vi "temperature control.vi"() -> ()   [LabVIEW 2026]
uses:
  <vilib>/Analysis/baseanly.llb/Mean (DBL).vi
  <vilib>/Instr/_visa.llb/VISA Configure Serial Port (Instr).vi
  <vilib>/Analysis/NI_AALBase.lvlib
panel:
  out "Event Log":string
  out "Alarm":bool
  out "Trend":cluster{dbl, "mean":dbl}(graph)
  out "Raw ADC":dbl
  out "Temperature °C":dbl(slide) scale=0.0..100.0
  in  "stop":bool
  in  "Log File Path":path=path "C:/Users/Anika Gupta/Desktop/temperature monitor/alarm_log.csv"
  in  "Averaging N":i32
  in  "High Limit":dbl
  in  "COM Port":refnum<visa-resource-name>
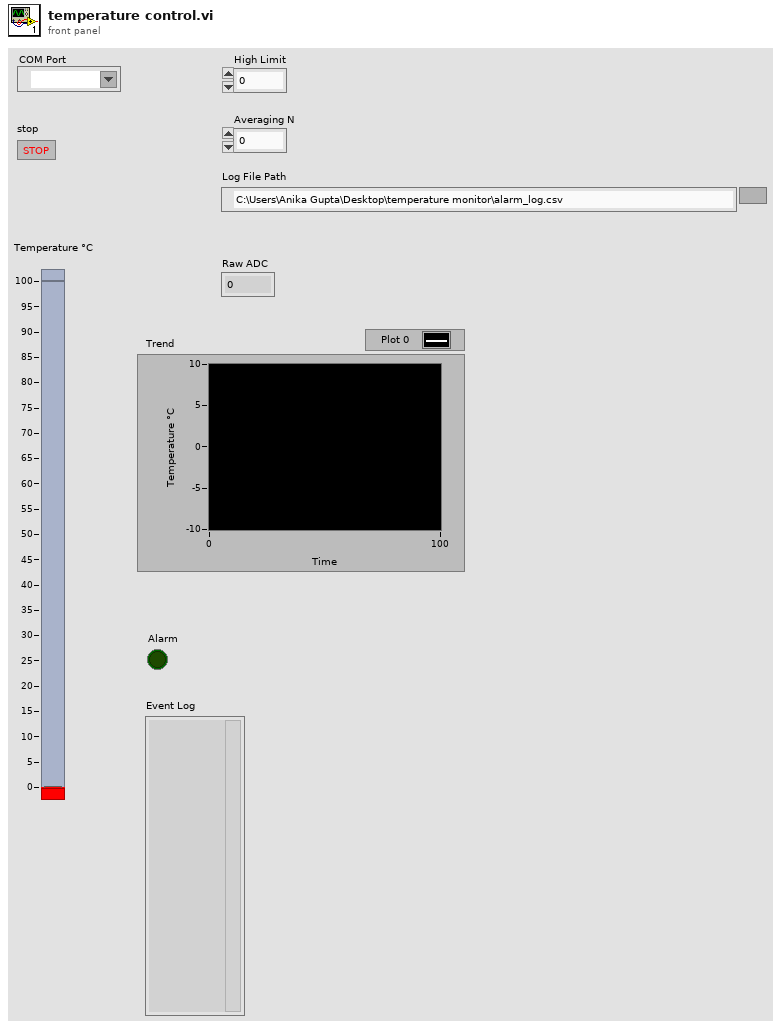
[diagram p1: front panel]
types:
  T1 = enum16{"open", "replace", "create", "open or create", "replace or create", "replace or create with confirmation"}
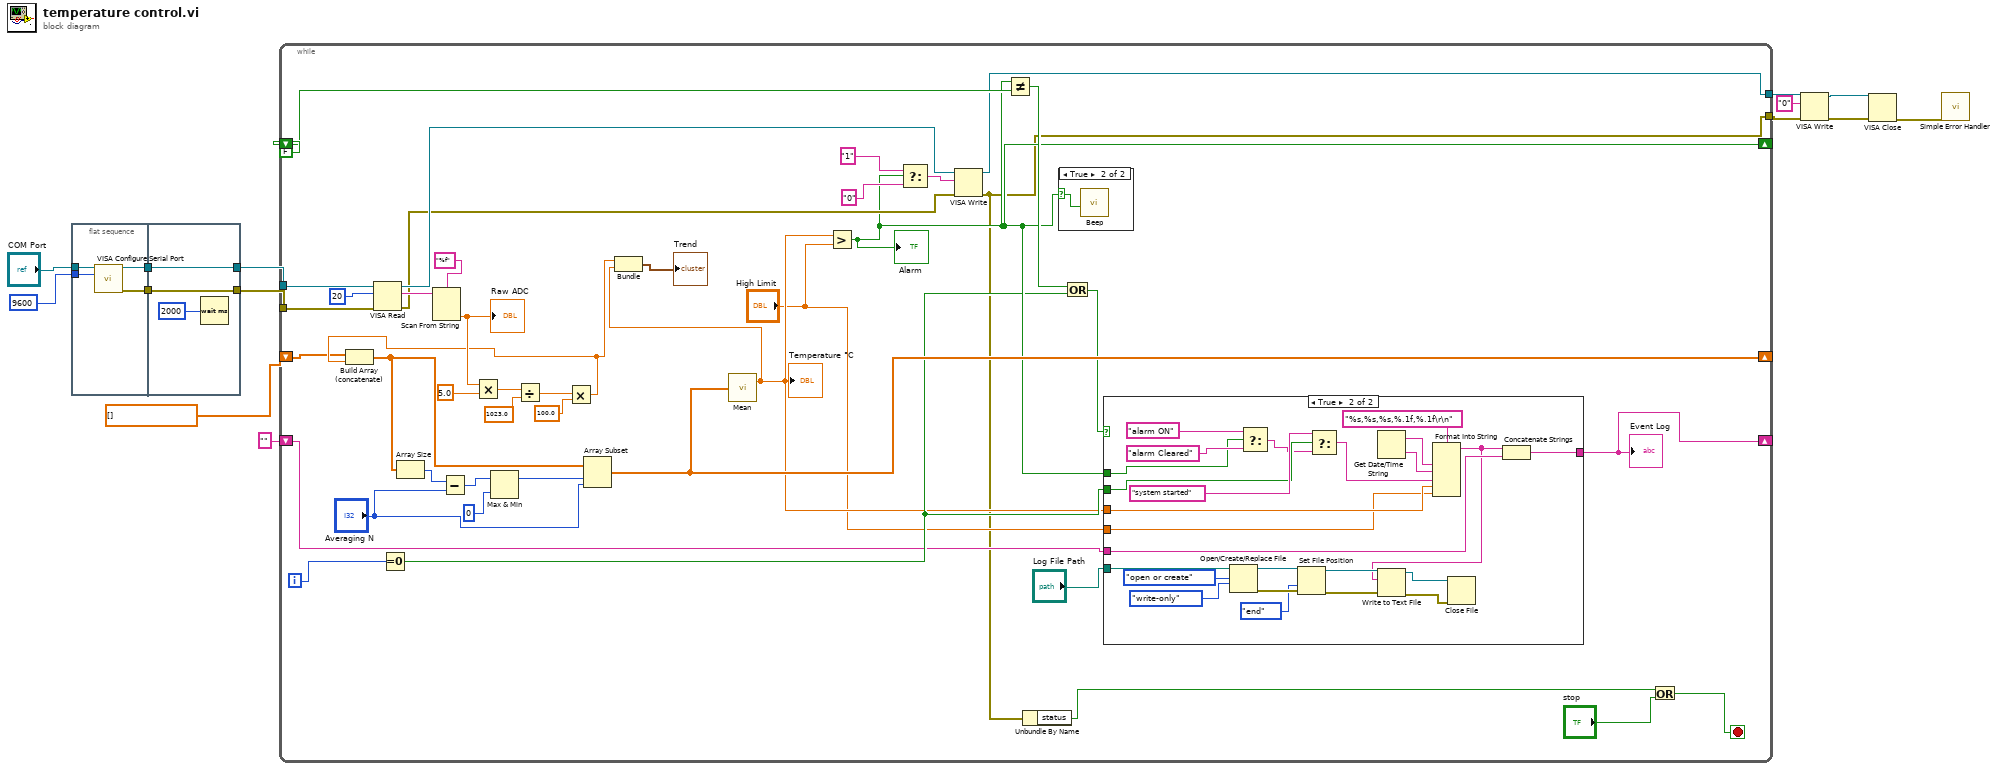
[diagram p0: block diagram]
diagram:
  n1 = flat-sequence {
    tunnel: "COM Port" -> [w19]
    tunnel: u32 9600 ("baud rate (9600)") -> [w18]
    tunnel: [w17] -> w13
    tunnel: [w16] -> w12
    tunnel: w13 -> [w21]
    tunnel: w12 -> [w20]
    tunnel: [w21] -> w11
    tunnel: [w20] -> w10
    frame #0 {
      n2 = call-poly "VISA Configure Serial Port"("VISA resource name"=w19, "baud rate (9600)"=w18) -> ("VISA resource name out"=w17:refnum<visa-resource-name>, "error out"=w16:errorcluster)  [unwired: 12 in]
    }
    frame #1 {
      n3 = Wait (ms)(milliseconds to wait=u32 2000) -> ()  [unwired: 1 out]
    }
  }
  n4 = while {
    tunnel: w11 -> [w64]
    tunnel: w10 -> [w63]
    shift-right: [w47] -> _
    shift-left: dbl[] [] -> [w23]
    shift-right: [w36] -> _
    shift-left: FALSE -> [w40]
    shift-right: [w32] -> _
    shift-left: "" -> [w31]
    tunnel: [w26] -> w6
    tunnel: [w25] -> w5
    i -> [w39]
    stop <- w27 stop-if-true
    n5 = VISA Read(VISA resource name=w64, byte count=u32 20, error in (no error)=w63) -> (VISA resource name out=w42:refnum<visa-resource-name>, read buffer=w61:string, error out=w41:errorcluster)  [unwired: 1 out]
    n6 = Equal To 0?(x=w39) -> (x = 0?=w35:bool)
    n7 = Scan From String(format string="%f", input string=w61) -> (output 1=w54:dbl)  [unwired: 3 in, 3 out]
    "Raw ADC" <- w54
    n8 = Multiply(x=w54, y=5.0) -> (x*y=w59:dbl)
    n9 = Divide(x=w59, y=1023.0) -> (x/y=w57:dbl)
    n10 = Multiply(x=w57, y=100.0) -> (x*y=w24:dbl)
    n11 = Build Array (concatenate)(w23, w24) -> (w50:dbl[])
    n12 = Array Size(array=w50) -> (size(s)=w53:i32)
    n13 = Subtract(x=w53, y="Averaging N") -> (x-y=w52:i32)
    n14 = Max & Min(x=w52, y=0) -> (max(x,y)=w49:i32)  [unwired: 1 out]
    n15 = Array Subset(array=w50, index=w49, length="Averaging N") -> (w47:dbl[])
    n16 = call-poly <vilib>:"Mean.vi"("X"=w47) -> ("mean"=w34:dbl)  [unwired: 1 out]
    "Temperature °C" <- w34
    n17 = Bundle(w24, "mean"=w34) -> (→"Trend":cluster{dbl, "mean":dbl})  [unwired: 1 in]
    n18 = Greater?(x=w34, y="High Limit") -> (0:w36:bool)
    "Alarm" <- w36
    n19 = Select(t="1", s=w36, f="0") -> (s? t:f=w43:string)
    n20 = VISA Write(VISA resource name=w42, write buffer=w43, error in (no error)=w41) -> (VISA resource name out=w26:refnum<visa-resource-name>, error out=w25:errorcluster)  [unwired: 1 out]
    n21 = Not Equal?(x=w36, y=w40) -> (x != y?=w38:bool)
    n22 = Unbundle By Name(w25) -> ("status"=w28:bool)
    n23 = case shown="True" w36 {
      selector: w36 -> [_ w91]
      frame False {
      }
      frame True {
        n24 = call <vilib>:"Beep.vi"("use system alert? (T)"=w91) -> ()  [unwired: 11 in]
      }
    }
    n25 = Or(x=w38, y=w35) -> (x .or. y?=w37:bool)
    n26 = case shown="True" w37 {
      tunnel: w36 -> [_ w86]
      tunnel: w35 -> [_ w87]
      tunnel: w34 -> [_ w81]
      tunnel: "High Limit" -> [_ w80]
      tunnel: [w65 w78] -> w32
      tunnel: w31 -> [w65 w77]
      tunnel: "Log File Path" -> [_ w76]
      frame False {
      }
      frame True {
        n27 = Open/Create/Replace File(file path (use dialog)=w76, operation (0:open)=T1."open or create", access (0:read/write)=enum16{"read/write", "read-only", "write-only"}."write-only") -> (refnum out=w73:refnum<file>, error out=w72:errorcluster)  [unwired: 3 in, 1 out]
        n28 = Select(t="alarm ON", s=w86, f="alarm Cleared") -> (s? t:f=w79:string)
        n29 = Set File Position(refnum=w73, from (0:start)=enum16{"start", "end", "current"}."end", error in=w72) -> (refnum out=w70:refnum<file>, error out=w69:errorcluster)  [unwired: 1 in]
        n30 = Select(t="system started", s=w87, f=w79) -> (s? t:f=w82:string)
        n31 = Get Date/Time String() -> (date string=w84:string, time string=w83:string)  [unwired: 3 in]
        n32 = Format Into String(format string="%s,%s,%s,%.1f,%.1f\r\n", w84, w83, w82, w81, w80) -> (resulting string=w68:string)  [unwired: 2 in, 1 out]
        n33 = Write to Text File(file (use dialog)=w70, text=w68, error in=w69) -> (refnum out=w67:refnum<file>, error out=w66:errorcluster)  [unwired: 1 in, 1 out]
        n34 = Close File(refnum=w67, error in=w66) -> ()  [unwired: 2 out]
        n35 = Concatenate Strings(w68, w77) -> (w78:string)
      }
    }
    "Event Log" <- w32
    n36 = Or(x=w28, y="stop") -> (x .or. y?=w27:bool)
  }
  n37 = VISA Write(VISA resource name=w6, write buffer="0", error in (no error)=w5) -> (VISA resource name out=w3:refnum<visa-resource-name>, error out=w2:errorcluster)  [unwired: 1 out]
  n38 = VISA Close(VISA resource name=w3, error in (no error)=w2) -> (error out=w1:errorcluster)
  n39 = call <vilib>:"Simple Error Handler.vi"("error in (no error)"=w1) -> ()  [unwired: 4 in, 5 out]
